vi "waitForInterrupt.vi"(6 "Debounce (us)":u32, 8 "error in (no error)":errorcluster, 9 "Timeout (ms)":i32=-1, 10 "Mode":T1, 11 "RPi Pin":T2) -> (0 "error out":errorcluster, 1 "TimeStamp (us)":u64, 2 "Detected":bool, 3 "RPi Pin out":T2, 4 "Detected Edge":T1=enum."Edge Falling")   [LabVIEW 2025, in "wiringPi.lvlib"]
doc: "/*\n * waitForInterrupt2:\n * Wait for Interrupt on a GPIO pin and use v2 of the character device API, need Kernel 5.1\n * Returns struct WPIWfiStatus\n *********************************************************************************\n */"
uses:
  wiringPi.lvlib
  Type Defs/GPIO Pins.ctl
  Type Defs/Edge Mode.ctl
  <vilib>/Utility/error.llb/Error Cluster From Error Code.vi
  <vilib>/ErrorRing/Error Ring.xnode
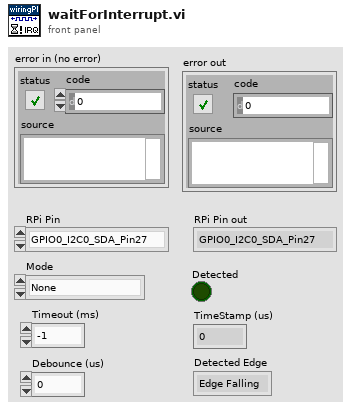
[diagram p1: front panel]
types:
  T1 = typedef "wiringPi.lvlib/Edge Mode.ctl" = enum32{"None", "Edge Falling", "Edge Rising", "Both"}
  T2 = typedef "wiringPi.lvlib/GPIO Pins.ctl" = enum32{"GPIO0_I2C0_SDA_Pin27", "GPIO1_I2C0_SDA1_Pin28", "GPIO2_I2C1_SDA_Pin3", "GPIO3_I2C1_SCL_Pin5", "GPIO4_GPCLK0_Pin7", "GPIO5_GPCLK1_Pin29", "GPIO6_GPCLK2_Pin31", "GPIO7_SPI_CE1_N_Pin26", "GPIO8_SPI_CE0_N_Pin24", "GPIO9_SPI0_MISO_Pin21", "GPIO10_SPI0_MOSI_Pin19", "GPIO11_SPI0_CLK_Pin23", "GPIO12_PWM0_Pin32", "GPIO13_PWM1_Pin33", "GPIO14_TXD0_Pin8", "GPIO15_RXD0_Pin10", "GPIO16_Pin36", "GPIO17_Pin11", "GPIO18_PWM0_Pin12", "GPIO19_PWM1_Pin35", "GPIO20_GPCLK0_Pin38", "GPIO21_GPCLK1_Pin40", "GPIO22_Pin15", "GPIO23_Pin16", "GPIO24_Pin18", "GPIO25_Pin22", "GPIO26_Pin37", "GPIO27_Pin13"}
  T3 = cluster{"statusOK":i32, "pinMCM":T2, "edge":T1, "ltimeStamp_us":u64}
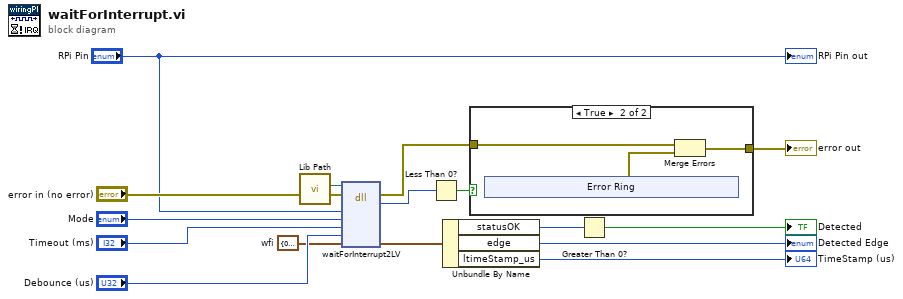
[diagram p0: block diagram]
diagram:
  w6 = T3 {"statusOK"=0, "pinMCM"=enum."GPIO16_Pin36", "edge"=enum."Both", "ltimeStamp_us"=3}  # wfi
  n1 = call "Lib Path.vi"() -> ("path out"=w1:path)  [unwired: 11 in]
  n2 = dll-call lib="libLVwiringPI.so" fn="waitForInterrupt2LV"(path in=w1, error in="error in (no error)", "pin"="RPi Pin", "edgemode"="Mode", "ms"="Timeout (ms)", "debounce_period_us"="Debounce (us)", "sfiStatus"=w6) -> (error out=w3:errorcluster, "return type"=w4:i64, "sfiStatus"=w7:T3)  [unwired: 5 in, 1 out]
  n3 = Less Than 0?(x=w4) -> (x < 0?=w2:bool)
  n4 = Unbundle By Name(w7) -> ("statusOK"=w5:i32, "edge"=→"Detected Edge":T1, "ltimeStamp_us"=→"TimeStamp (us)":u64)
  n5 = case shown="True" w2 {
    tunnel: w3 -> [w17 w19]
    tunnel: [w17 w20] -> w8
    frame False {
    }
    frame True {
      n6 = xnode "Error Ring"() -> ("error out"=w18:errorcluster)
      n7 = Merge Errors(w19, w18) -> (w20:errorcluster)
    }
  }
  "error out" <- w8
  n8 = Greater Than 0?(x=w5) -> (x > 0?=→"Detected":bool)
  "RPi Pin out" <- "RPi Pin"
